vi "_testNewFile(AIM).vi"() -> ()   [LabVIEW 2020]
uses:
  Source/Libraries/Aim_Parameter_ni/_tyedefs/label_type.ctl
  Source/Libraries/Aim_Parameter_ni/_tyedefs/parameter_type.ctl
  Source/Libraries/Aim_Parameter_ni/AIM_Parameter_ni.lvlib
panel:
  in  "parameter configuration":T1
  in  "label configuration":T2 {"sdi" items=["All", "Item00", "Item01", "Item10", "Item11"]}
  in  "speed (high)":i32(ring) items=["high", "low"]
  in  "direction (incoming)":i32(ring) items=["incoming", "outgoing"]
  in  "hardwareChannel":i32
  out "SerializeXML":bool
  out "error out":errorcluster
  in  "XML path":path=path "C:/Users/Administrator/Desktop/GIT/Ballard-Arinc-429-XML-Generator/Database Examples/ParametersAIM.xml"
  in  "mode (Create)":i32(ring)=2 items=["CreateNew"=1, "Create"=2, "Open"=3, "OpenOrCreate"=4, "Truncate"=5, "Append"=6]
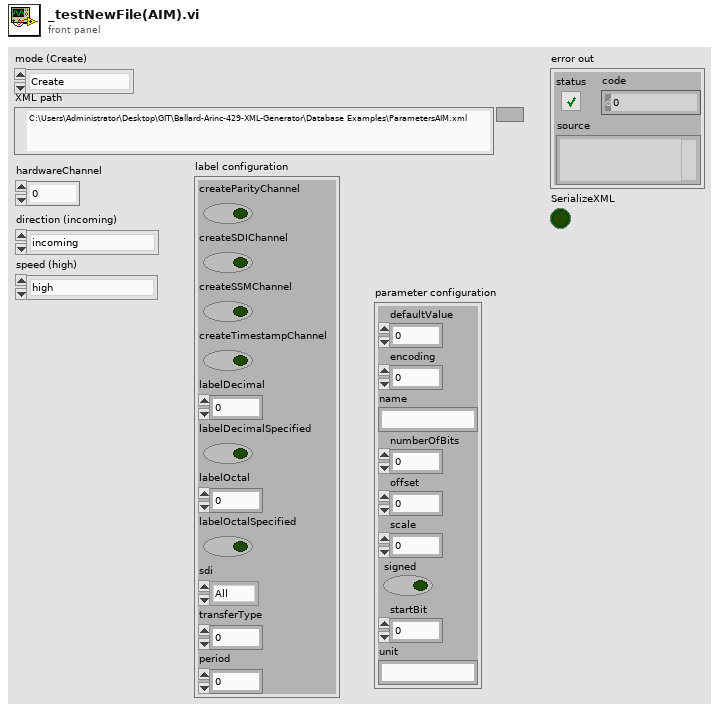
[diagram p1: front panel]
types:
  T1 = typedef "AIM_Parameter_ni.lvlib/parameter_type.ctl" = cluster{"defaultValue":dbl, "encoding":i32, "name":string, "numberOfBits":i32, "offset":dbl, "scale":dbl, "signed":bool, "startBit":i32, "unit":string}
  T2 = typedef "AIM_Parameter_ni.lvlib/label_type.ctl" = cluster{"createParityChannel":bool, "createSDIChannel":bool, "createSSMChannel":bool, "createTimestampChannel":bool, "labelDecimal":i32, "labelDecimalSpecified":bool, "labelOctal":i32, "labelOctalSpecified":bool, "sdi":i32, "transferType":i32, "period":i32}
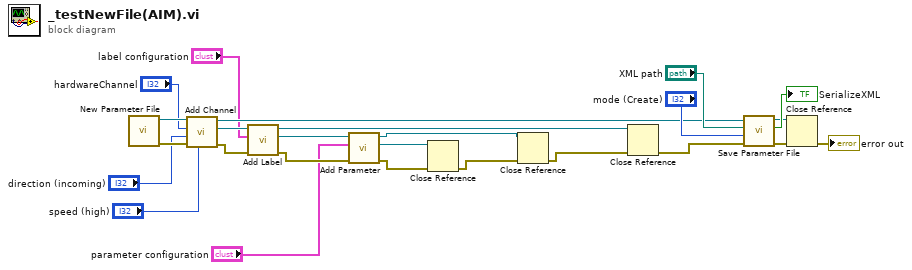
[diagram p0: block diagram]
diagram:
  n1 = call "New Parameter File.vi"() -> ("error out"=w18:errorcluster, "new parameter file"=w19:refnum<k24>)  [unwired: 10 in]
  n2 = call "Add Channel.vi"("speed (high)"="speed (high)", "error in"=w18, "direction (incoming)"="direction (incoming)", "hardwareChannel"="hardwareChannel", "parameter file in"=w19) -> ("error out"=w11:errorcluster, "new channel"=w12:refnum<k24>, "parameter file out"=w17:refnum<k24>)  [unwired: 4 in]
  n3 = call "Add Label.vi"("error in"=w11, "label configuration"="label configuration", "channel in"=w12) -> ("error out"=w2:errorcluster, "new label"=w7:refnum<k24>, "channel out"=w10:refnum<k24>)  [unwired: 6 in]
  n4 = call "Add Parameter.vi"("error in"=w2, "parameter configuration"="parameter configuration", "label in"=w7) -> ("error out"=w5:errorcluster, "new parameter"=w6:refnum<k24>, "label out"=w4:refnum<k24>)  [unwired: 6 in]
  n5 = Close Reference(reference=w6, error in (no error)=w5) -> (error out=w3:errorcluster)
  n6 = Close Reference(reference=w4, error in (no error)=w3) -> (error out=w9:errorcluster)
  n7 = Close Reference(reference=w10, error in (no error)=w9) -> (error out=w16:errorcluster)
  n8 = call "Save Parameter File.vi"("error in"=w16, "mode (Create)"="mode (Create)", "XML path"="XML path", "parameter file in"=w17) -> ("error out"=w23:errorcluster, "SerializeXML"=→"SerializeXML":bool, "parameter file out"=w20:refnum<k24>)  [unwired: 5 in]
  n9 = Close Reference(reference=w20, error in (no error)=w23) -> (error out=→"error out":errorcluster)
